vi "Draw Trajectory.vi"(7 "Robot Index":i32, 8 "Hide Path":bool, 9 "new picture in":picture, 10 "Trajectory Data":T1, 11 "Picture in":refnum<vi>) -> (0 "Path Points":cluster{"x":dbl, "y":dbl}[](array[cluster]), 2 "Output Point":T3, 3 "new picture":picture)   [LabVIEW 2023]
uses:
  Types/Trajectory Data.ctl
  Types/Segment Type.ctl
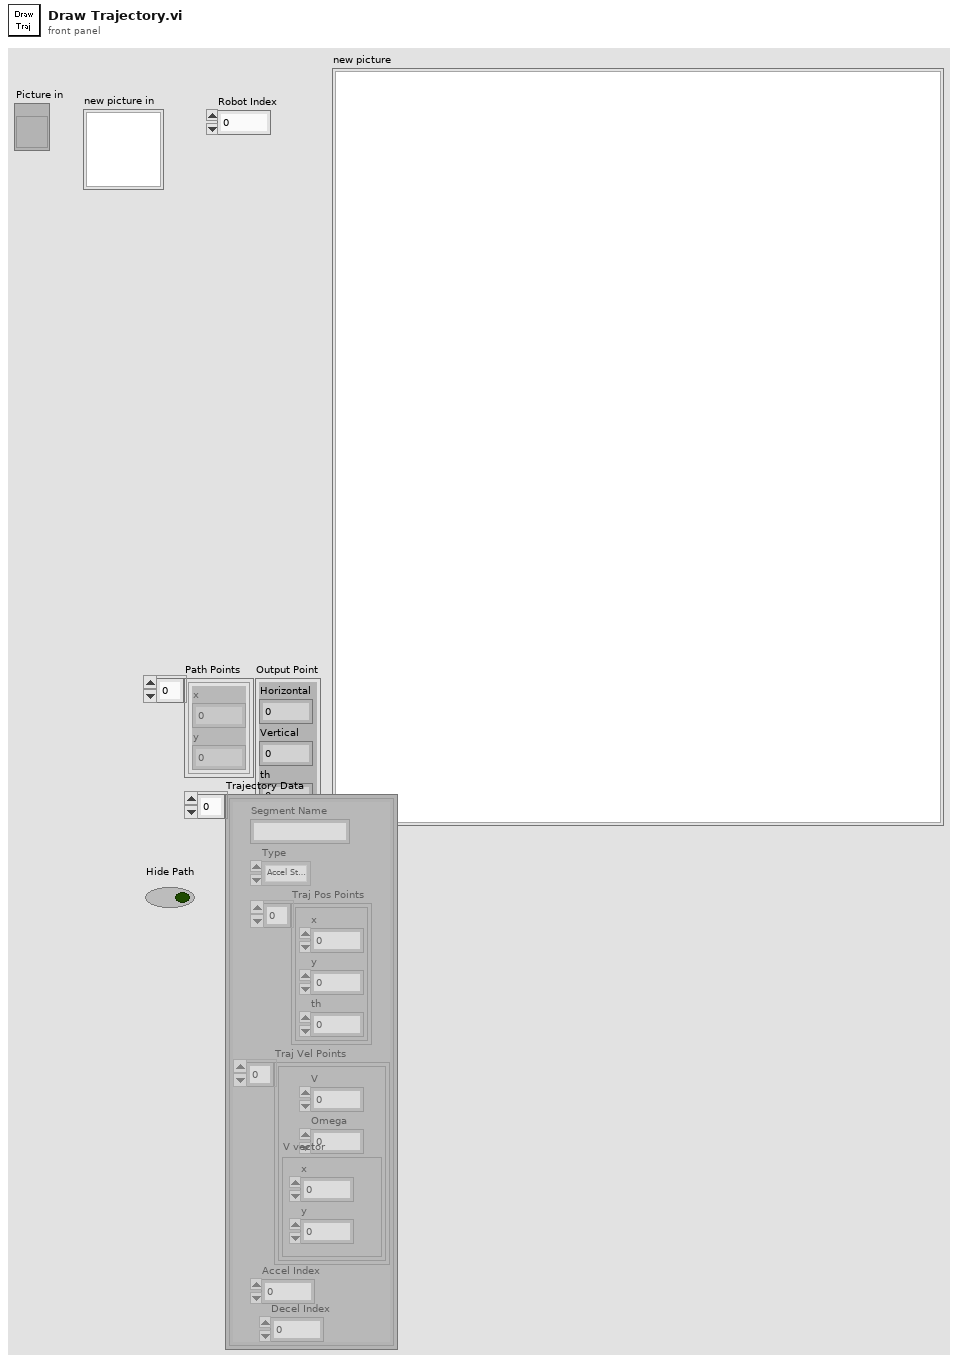
[diagram p1: front panel]
types:
  T1 = typedef "Trajectory Data.ctl" = cluster{"Segment Name":string, "Type":T2, "Traj Pos Points":cluster{"x":dbl, "y":dbl, "th":dbl}[], "Traj Vel Points":cluster{"V":dbl, "Omega":dbl, "V vector":cluster{"y":dbl, "x":dbl}}[], "Accel Index":i32, "Decel Index":i32}[]
  T2 = typedef "Segment Type.ctl" = enum16{"Accel Straight", "Const Straight", "Blend", "Circle", "Bezier"}
  T3 = cluster{"Horizontal":dbl, "Vertical":dbl, "th":dbl}
  T4 = cluster{"Width":u16, "Style":enum32{"Solid", "Dash", "Dot", "DashDot", "DashDotDot"}}
  T5 = typedef "LVPositionTypeDef.ctl" = cluster{"Left":i32, "Top":i32}
  T6 = typedef "LVBoundsTypeDef.ctl" = cluster{"Width":u32, "Height":u32}
  T7 = cluster{"V":dbl, "Omega":dbl, "V vector":cluster{"y":dbl, "x":dbl}}[]
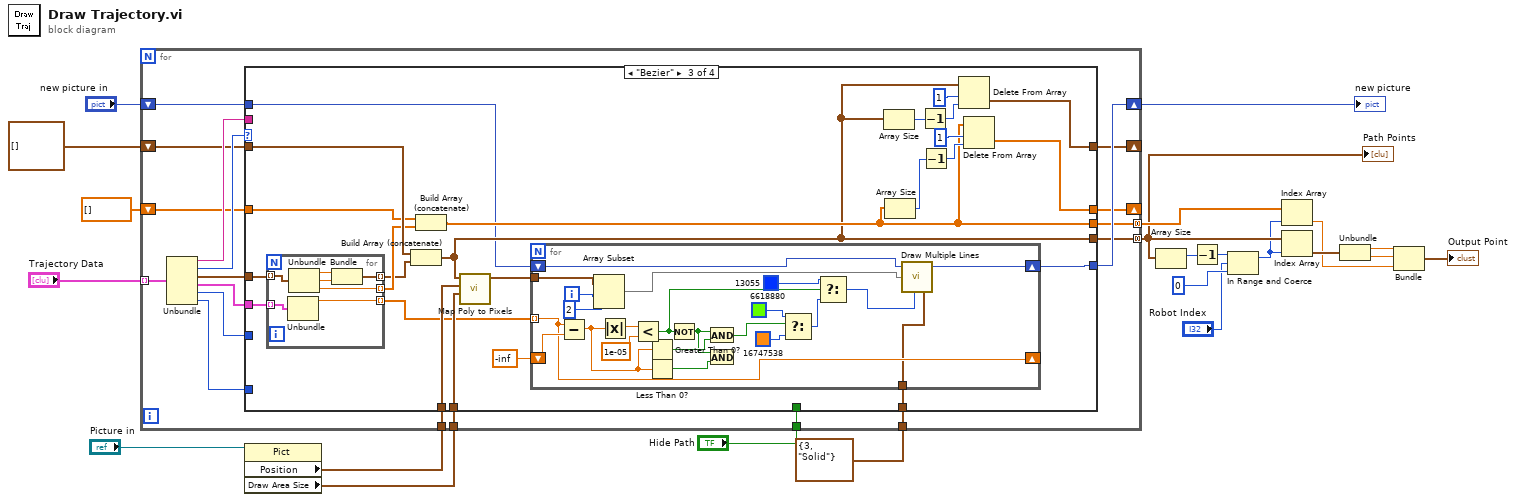
[diagram p0: block diagram]
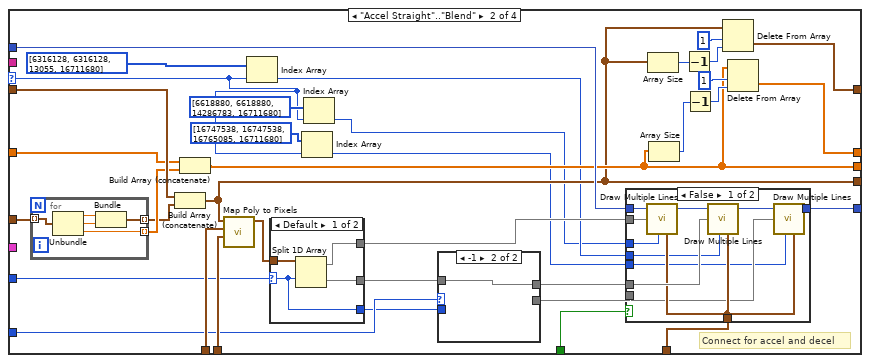
[diagram p3: hidden frame]
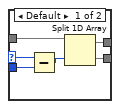
[diagram p5: hidden frame]
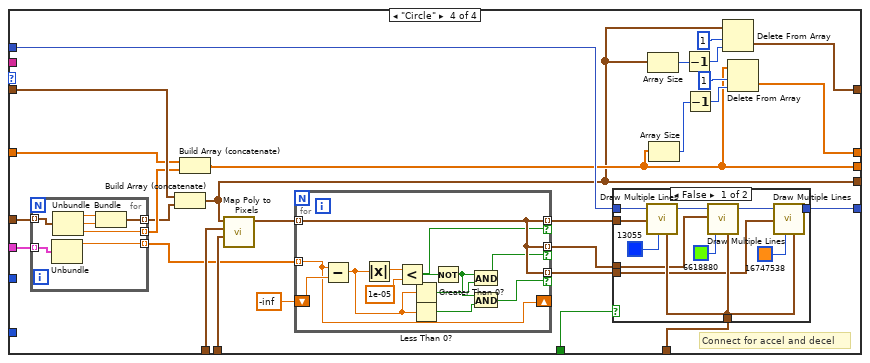
[diagram p7: hidden frame]
diagram:
  n1 = property on="Property Node" class="Pict"(reference="Picture in") -> ("Position"=w18:T5, "Draw Area Size"=w19:T6)  [unwired: 1 in, 2 out]
  n2 = for {
    tunnel: "Trajectory Data" -> [w41] mode=indexing
    shift-right: [w34] -> w17
    shift-left: "new picture in" -> [w33]
    tunnel: T4 {"Width"=3, "Style"=enum."Solid"} ("pen") -> [w37]
    tunnel: w19 -> [w36]
    tunnel: w18 -> [w35]
    tunnel: [w31] -> w10 mode=concatenating
    tunnel: [w30] -> w11 mode=concatenating
    shift-right: [w28] -> _
    shift-left: cluster{"x":dbl, "y":dbl}[] [] -> [w27]
    shift-right: [w26] -> _
    shift-left: dbl[] [] -> [w25]
    tunnel: "Hide Path" -> [w23]
    n3 = Unbundle(w41) -> ("Segment Name"=w40:string, "Type"=w32:T2, "Traj Pos Points"=w39:cluster{"x":dbl, "y":dbl, "th":dbl}[], "Traj Vel Points"=w38:T7, "Accel Index"=w29:i32, "Decel Index"=w24:i32)
    n4 = case shown="\"Bezier\"" w32 {
      selector: w32 -> [_ w48 _ _]
      tunnel: w40 -> [_ _ _ _]
      tunnel: w39 -> [_ w80 w133 w190]
      tunnel: w38 -> [_ _ w116 w169]
      tunnel: w37 -> [_ w59 w112 w173]
      tunnel: w36 -> [_ w79 w132 w189]
      tunnel: w35 -> [_ w77 w131 w187]
      tunnel: [w44 w60 w110 w174] -> w34
      tunnel: w33 -> [w44 w78 w111 w188]
      tunnel: [_ w54 w117 w171] -> w31
      tunnel: [_ w66 w121 w177] -> w30
      tunnel: w29 -> [_ w63 _ _]
      tunnel: [w43 w71 w126 w182] -> w28
      tunnel: w27 -> [w43 w74 w129 w185]
      tunnel: [w42 w67 w122 w178] -> w26
      tunnel: w25 -> [w42 w64 w119 w175]
      tunnel: w24 -> [_ w62 _ _]
      tunnel: w23 -> [_ w45 _ w170]
      frame Default {
      }
      frame "Accel Straight".."Blend" {
        # "Connect for accel and decel"
        n5 = for {
          tunnel: w80 -> [w109] mode=indexing
          tunnel: [w108] -> w55 mode=indexing
          tunnel: [w105] -> w65 mode=indexing
          n6 = Unbundle(w109) -> ("x"=w107:dbl, "y"=w106:dbl, "th"=w105:dbl)
          n7 = Bundle("x"=w107, "y"=w106) -> (w108:cluster{"x":dbl, "y":dbl})  [unwired: 1 in]
        }
        n8 = Build Array (concatenate)(w74, w55) -> (w54:cluster{"x":dbl, "y":dbl}[])
        n9 = Build Array (concatenate)(w64, w65) -> (w66:dbl[])
        n10 = call "Map Poly to Pixels.vi"("Draw Area Size"=w79, "Position"=w77, "Coords"=w54) -> ("Coords"=w53:cluster{"Horizontal":dbl, "Vertical":dbl}[])  [unwired: 8 in]
        n11 = Index Array(array=u32[] [6316128, 6316128, 13055, 16711680], index=w48) -> (element=w51:u32)
        n12 = case shown="Default" w63 {
          selector: w63 -> [w100 _]
          tunnel: w53 -> [w103 w104]
          tunnel: [w101 _] -> w52
          tunnel: [w102 w104] -> w57
          tunnel: [w100 _] -> w56
          frame Default {
            n13 = Split 1D Array(array=w103, index=w100) -> (first subarray=w101:cluster{"Horizontal":dbl, "Vertical":dbl}[], second subarray=w102:cluster{"Horizontal":dbl, "Vertical":dbl}[])
          }
          frame -1 {
          }
        }
        n14 = Index Array(array=u32[] [16747538, 16747538, 16765085, 16711680], index=w48) -> (element=w46:u32)
        n15 = Index Array(array=u32[] [6618880, 6618880, 14286783, 16711680], index=w48) -> (element=w47:u32)
        n16 = case shown="-1" w62 {
          selector: w62 -> [w95 _]
          tunnel: w57 -> [w98 w99]
          tunnel: [w97 w99] -> w61
          tunnel: [w96 _] -> w58
          tunnel: w56 -> [w94 _]
          frame Default {
            n17 = Subtract(x=w95, y=w94) -> (x-y=w93:i32)
            n18 = Split 1D Array(array=w98, index=w93) -> (first subarray=w97:cluster{"Horizontal":dbl, "Vertical":dbl}[], second subarray=w96:cluster{"Horizontal":dbl, "Vertical":dbl}[])
          }
          frame -1 {
          }
        }
        n19 = case shown="False" w45 {
          tunnel: w78 -> [w91 w92]
          tunnel: w61 -> [w89 _]
          tunnel: [w87 w92] -> w60
          tunnel: w59 -> [w86 _]
          tunnel: w58 -> [w85 _]
          tunnel: w52 -> [w84 _]
          tunnel: w51 -> [w83 _]
          tunnel: w47 -> [w82 _]
          tunnel: w46 -> [w81 _]
          frame False {
            n20 = call <vilib>:"Draw Multiple Lines.vi"("picture"=w91, "line endpoints"=w84, "color(black)"=w82, "pen"=w86) -> ("new picture"=w90:picture)  [unwired: 5 in]
            n21 = call <vilib>:"Draw Multiple Lines.vi"("picture"=w90, "line endpoints"=w89, "color(black)"=w83, "pen"=w86) -> ("new picture"=w88:picture)  [unwired: 5 in]
            n22 = call <vilib>:"Draw Multiple Lines.vi"("picture"=w88, "line endpoints"=w85, "color(black)"=w81, "pen"=w86) -> ("new picture"=w87:picture)  [unwired: 5 in]
          }
          frame True {
          }
        }
        n23 = Array Size(array=w54) -> (size(s)=w75:i32)
        n24 = Array Size(array=w66) -> (size(s)=w68:i32)
        n25 = Decrement(x=w75) -> (x-1=w72:i32)
        n26 = Decrement(x=w68) -> (x-1=w70:i32)
        n27 = Delete From Array(array=w54, length=1, index=w72) -> (deleted portion=w71:cluster{"x":dbl, "y":dbl}[])  [unwired: 1 out]
        n28 = Delete From Array(array=w66, length=1, index=w70) -> (deleted portion=w67:dbl[])  [unwired: 1 out]
      }
      frame "Bezier" {
        n29 = for {
          tunnel: w133 -> [w162] mode=indexing
          tunnel: [w161] -> w118 mode=indexing
          tunnel: [w158] -> w120 mode=indexing
          tunnel: w116 -> [w157] mode=indexing
          tunnel: [w156] -> w114 mode=indexing
          n30 = Unbundle(w157) -> ("V"=w156:dbl)  [unwired: 2 out]
          n31 = Unbundle(w162) -> ("x"=w160:dbl, "y"=w159:dbl, "th"=w158:dbl)
          n32 = Bundle("x"=w160, "y"=w159) -> (w161:cluster{"x":dbl, "y":dbl})  [unwired: 1 in]
        }
        n33 = Build Array (concatenate)(w129, w118) -> (w117:cluster{"x":dbl, "y":dbl}[])
        n34 = Build Array (concatenate)(w119, w120) -> (w121:dbl[])
        n35 = call "Map Poly to Pixels.vi"("Draw Area Size"=w132, "Position"=w131, "Coords"=w117) -> ("Coords"=w115:cluster{"Horizontal":dbl, "Vertical":dbl}[])  [unwired: 8 in]
        n36 = for {
          tunnel: w115 -> [w135]
          tunnel: w114 -> [w152] mode=indexing
          shift-right: [w152] -> _
          shift-left: -inf -> [w155]
          tunnel: w112 -> [w140]
          shift-right: [w138] -> w110
          shift-left: w111 -> [w139]
          i -> [w137]
          n37 = Subtract(x=w152, y=w155) -> (x-y=w150:dbl)
          n38 = Array Subset(array=w135, index=w137, length=2) -> (w134:cluster{"Horizontal":dbl, "Vertical":dbl}[])
          n39 = Absolute Value(x=w150) -> (abs(x)=w154:dbl)
          n40 = Less?(x=w154, y=1e-05) -> (x < y?=w146:bool)
          n41 = Greater Than 0?(x=w150) -> (x > 0?=w151:bool)
          n42 = Less Than 0?(x=w150) -> (x < 0?=w149:bool)
          n43 = Not(x=w146) -> (.not. x?=w148:bool)
          n44 = And(x=w148, y=w151) -> (x .and. y?=w147:bool)
          n45 = And(x=w148, y=w149) -> ()  [unwired: 1 out]
          n46 = Select(t=u32 6618880 ("color(black)"), s=w147, f=u32 16747538 ("color(black)")) -> (s? t:f=w144:u32)
          n47 = Select(t=u32 13055 ("color(black)"), s=w146, f=w144) -> (s? t:f=w141:u32)
          n48 = call <vilib>:"Draw Multiple Lines.vi"("picture"=w139, "line endpoints"=w134, "color(black)"=w141, "pen"=w140) -> ("new picture"=w138:picture)  [unwired: 5 in]
        }
        n49 = Array Size(array=w117) -> (size(s)=w130:i32)
        n50 = Array Size(array=w121) -> (size(s)=w123:i32)
        n51 = Decrement(x=w130) -> (x-1=w127:i32)
        n52 = Decrement(x=w123) -> (x-1=w125:i32)
        n53 = Delete From Array(array=w117, length=1, index=w127) -> (deleted portion=w126:cluster{"x":dbl, "y":dbl}[])  [unwired: 1 out]
        n54 = Delete From Array(array=w121, length=1, index=w125) -> (deleted portion=w122:dbl[])  [unwired: 1 out]
      }
      frame "Circle" {
        # "Connect for accel and decel"
        n55 = for {
          tunnel: w190 -> [w221] mode=indexing
          tunnel: [w220] -> w172 mode=indexing
          tunnel: [w217] -> w176 mode=indexing
          tunnel: w169 -> [w216] mode=indexing
          tunnel: [w215] -> w167 mode=indexing
          n56 = Unbundle(w216) -> ("V"=w215:dbl)  [unwired: 2 out]
          n57 = Unbundle(w221) -> ("x"=w219:dbl, "y"=w218:dbl, "th"=w217:dbl)
          n58 = Bundle("x"=w219, "y"=w218) -> (w220:cluster{"x":dbl, "y":dbl})  [unwired: 1 in]
        }
        n59 = Build Array (concatenate)(w185, w172) -> (w171:cluster{"x":dbl, "y":dbl}[])
        n60 = Build Array (concatenate)(w175, w176) -> (w177:dbl[])
        n61 = call "Map Poly to Pixels.vi"("Draw Area Size"=w189, "Position"=w187, "Coords"=w171) -> ("Coords"=w168:cluster{"Horizontal":dbl, "Vertical":dbl}[])  [unwired: 8 in]
        n62 = for {
          tunnel: w168 -> [w199] mode=indexing
          tunnel: w167 -> [w198] mode=indexing
          shift-right: [w198] -> _
          shift-left: -inf -> [w202]
          tunnel: [w199] -> w165 mode=indexing if=w193
          tunnel: [w199] -> w164 mode=indexing if=w192
          tunnel: [w199] -> w163 mode=indexing if=w191
          n63 = Subtract(x=w198, y=w202) -> (x-y=w196:dbl)
          n64 = Absolute Value(x=w196) -> (abs(x)=w201:dbl)
          n65 = Less?(x=w201, y=1e-05) -> (x < y?=w193:bool)
          n66 = Greater Than 0?(x=w196) -> (x > 0?=w197:bool)
          n67 = Less Than 0?(x=w196) -> (x < 0?=w195:bool)
          n68 = Not(x=w193) -> (.not. x?=w194:bool)
          n69 = And(x=w194, y=w197) -> (x .and. y?=w192:bool)
          n70 = And(x=w194, y=w195) -> (x .and. y?=w191:bool)
        }
        n71 = case shown="False" w170 {
          tunnel: w188 -> [w213 w214]
          tunnel: [w210 w214] -> w174
          tunnel: w173 -> [w209 _]
          tunnel: w165 -> [w206 _]
          tunnel: w164 -> [w205 _]
          tunnel: w163 -> [w204 _]
          frame False {
            n72 = call <vilib>:"Draw Multiple Lines.vi"("picture"=w213, "line endpoints"=w206, "color(black)"=u32 13055, "pen"=w209) -> ("new picture"=w212:picture)  [unwired: 5 in]
            n73 = call <vilib>:"Draw Multiple Lines.vi"("picture"=w212, "line endpoints"=w205, "color(black)"=u32 6618880, "pen"=w209) -> ("new picture"=w211:picture)  [unwired: 5 in]
            n74 = call <vilib>:"Draw Multiple Lines.vi"("picture"=w211, "line endpoints"=w204, "color(black)"=u32 16747538, "pen"=w209) -> ("new picture"=w210:picture)  [unwired: 5 in]
          }
          frame True {
          }
        }
        n75 = Array Size(array=w171) -> (size(s)=w186:i32)
        n76 = Array Size(array=w177) -> (size(s)=w179:i32)
        n77 = Decrement(x=w186) -> (x-1=w183:i32)
        n78 = Decrement(x=w179) -> (x-1=w181:i32)
        n79 = Delete From Array(array=w171, length=1, index=w183) -> (deleted portion=w182:cluster{"x":dbl, "y":dbl}[])  [unwired: 1 out]
        n80 = Delete From Array(array=w177, length=1, index=w181) -> (deleted portion=w178:dbl[])  [unwired: 1 out]
      }
    }
  }
  "new picture" <- w17
  "Path Points" <- w10
  n81 = Array Size(array=w10) -> (size(s)=w9:i32)
  n82 = Decrement(x=w9) -> (x-1=w8:i32)
  n83 = In Range and Coerce(upper limit=w8, x="Robot Index", lower limit=u16 0 ("Width")) -> (coerced(x)=w5:i32)  [unwired: 1 out]
  n84 = Index Array(array=w11, index=w5) -> (element=w13:dbl)
  n85 = Index Array(array=w10, index=w5) -> (element=w16:cluster{"x":dbl, "y":dbl})
  n86 = Unbundle(w16) -> ("x"=w15:dbl, "y"=w14:dbl)
  n87 = Bundle("x"=w15, "y"=w14, "th"=w13) -> (→"Output Point":cluster{"x":dbl, "y":dbl, "th":dbl})  [unwired: 1 in]
